vi "batch-averager-deep.vi"() -> ()   [LabVIEW 2026]
doc: "Classic LabVIEW state machine in the NI canonical form (as exported from examples/Design Patterns/State Machine/State Machine Fundamentals.vi): an inline enum type uint16{Init,Load,Accumulate,Report,Stop} carries the state through a shift register; a Case Structure inside a While loop selects the frame by that state; each frame computes the next state (a constant, or a Select between two state constants when the transition is conditional) and writes every data register through a per-frame case Out tunnel, which is the per-state multiplexer for the register value. The Stop frame is the only one that raises the stop flag through a conditional (cond=true) tunnel wired straight to the loop condition. States: Init resets the registers; Load takes the next item from Items; Accumulate adds it to the sum, advances the index and branches back to Load or on to Report by comparing the index against the item count; Report divides sum by count into the average; Stop ends the loop. Every visited state is appended to a transition Log string register. Initial State accepts any state item so the machine can start mid-sequence."
panel:
  out "Log":string
  out "Average":dbl
  out "Items Processed":i32
  out "Sum":dbl
  out "Final State":T1(ring)
  in  "Items":dbl[](array[numeric])=[1.5, 2.5, 3.5, 4.5]
  in  "Initial State":T1(ring)
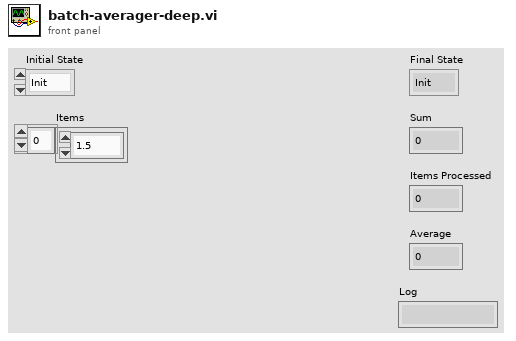
[diagram p1: front panel]
types:
  T1 = enum16{"Init", "Load", "Accumulate", "Report", "Stop"}
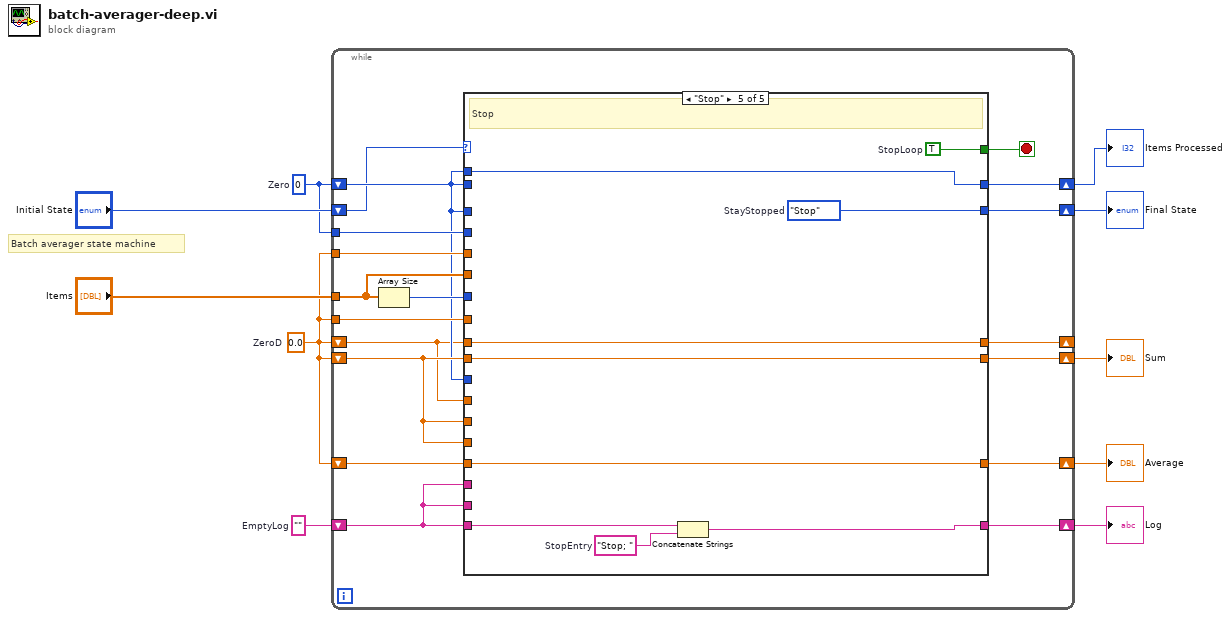
[diagram p0: block diagram]
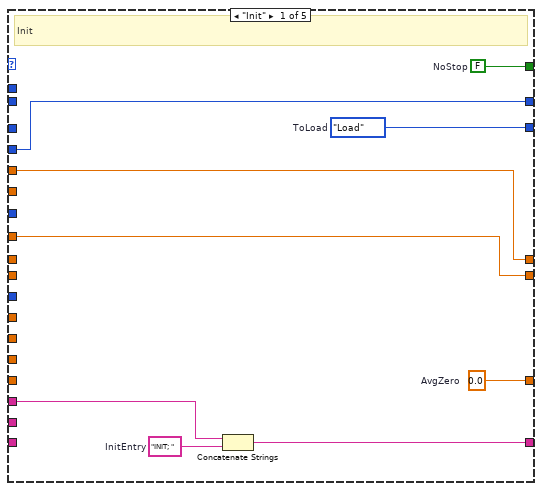
[diagram p2: hidden frame]
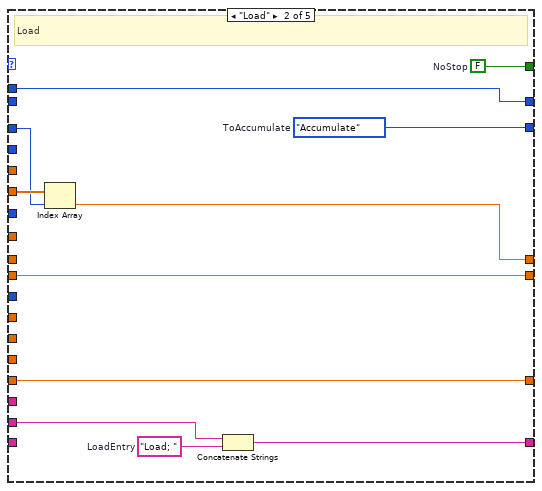
[diagram p3: hidden frame]
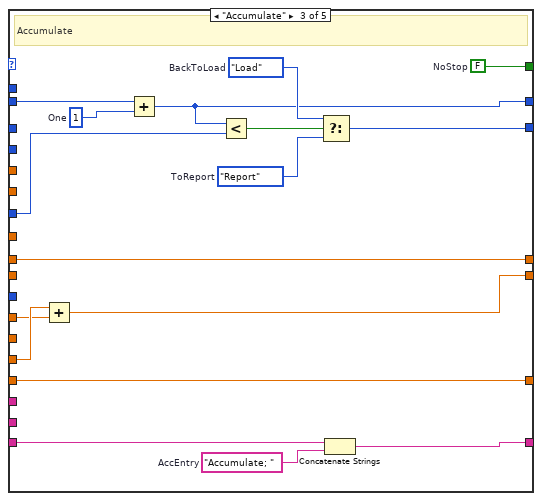
[diagram p4: hidden frame]
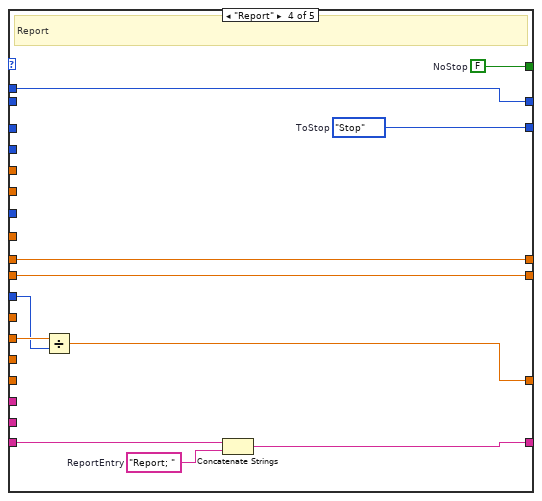
[diagram p5: hidden frame]
diagram:
  w8 = ""  # EmptyLog
  w6 = 0.0  # ZeroD
  w7 = 0  # Zero
  # "Batch averager state machine"
  n1 = while {
    tunnel: "Items" -> [w18]
    shift-right: [w28] -> w5
    shift-left: "Initial State" -> [w11]
    shift-right: [w26] -> w4
    shift-left: w6 -> [w15]
    shift-right: [w25] -> w3
    shift-left: w7 -> [w14]
    shift-right: [w24] -> _
    shift-left: w6 -> [w13]
    shift-right: [w23] -> w1
    shift-left: w8 -> [w16]
    shift-right: [w22] -> w2
    shift-left: w6 -> [w12]
    tunnel: w6 -> [w21]
    tunnel: w7 -> [w20]
    tunnel: w6 -> [w19]
    stop <- w27 stop-if-true
    n2 = Array Size(array=w18) -> (size(s)=w17:i32)
    n3 = case shown="\"Stop\"" w11 {
      tunnel: [w37 w46 w57 w74 w85] -> w28
      tunnel: [w36 w45 w56 w73 w84] -> w27
      tunnel: [w32 w41 w52 w69 w80] -> w26
      tunnel: [w31 w40 w51 w68 w79] -> w25
      tunnel: [w30 w39 w50 w67 w78] -> w24
      tunnel: [w33 w42 w53 w70 w81] -> w23
      tunnel: [w29 w38 w49 w66 w77] -> w22
      tunnel: w16 -> [w35 _ _ _ _]
      tunnel: w21 -> [w32 _ _ _ _]
      tunnel: w20 -> [w31 _ _ _ _]
      tunnel: w19 -> [w30 _ _ _ _]
      tunnel: w18 -> [_ w48 _ _ _]
      tunnel: w14 -> [_ w47 _ _ _]
      tunnel: w16 -> [_ w44 _ _ _]
      tunnel: w15 -> [_ _ w65 _ _]
      tunnel: w13 -> [_ _ w64 _ _]
      tunnel: w14 -> [_ _ w63 _ _]
      tunnel: w17 -> [_ _ w61 _ _]
      tunnel: w15 -> [_ _ _ w76 _]
      tunnel: w14 -> [_ _ _ w75 _]
      tunnel: w16 -> [_ _ w55 w72 w83]
      tunnel: w15 -> [_ w41 _ w69 w80]
      tunnel: w14 -> [_ w40 _ w68 w79]
      tunnel: w13 -> [_ _ w50 w67 w78]
      tunnel: w12 -> [_ w38 w49 _ w77]
      frame "Init" {
        w29 = 0.0  # AvgZero
        w34 = "INIT; "  # InitEntry
        w36 = FALSE  # NoStop
        w37 = T1."Load"  # ToLoad
        # "Init"
        n4 = Concatenate Strings(w35, w34) -> (w33:string)
      }
      frame "Load" {
        w43 = "Load; "  # LoadEntry
        w45 = FALSE  # NoStop
        w46 = T1."Accumulate"  # ToAccumulate
        # "Load"
        n5 = Index Array(array=w48, index=w47) -> (element=w39:dbl)
        n6 = Concatenate Strings(w44, w43) -> (w42:string)
      }
      frame "Accumulate" {
        w54 = "Accumulate; "  # AccEntry
        w56 = FALSE  # NoStop
        w58 = T1."Report"  # ToReport
        w60 = T1."Load"  # BackToLoad
        w62 = 1  # One
        # "Accumulate"
        n7 = Add(x=w65, y=w64) -> (x+y=w52:dbl)
        n8 = Add(x=w63, y=w62) -> (x+y=w51:i32)
        n9 = Less?(x=w51, y=w61) -> (x < y?=w59:bool)
        n10 = Select(t=w60, s=w59, f=w58) -> (s? t:f=w57:T1)
        n11 = Concatenate Strings(w55, w54) -> (w53:string)
      }
      frame "Report" {
        w71 = "Report; "  # ReportEntry
        w73 = FALSE  # NoStop
        w74 = T1."Stop"  # ToStop
        # "Report"
        n12 = Divide(x=w76, y=w75) -> (x/y=w66:dbl)
        n13 = Concatenate Strings(w72, w71) -> (w70:string)
      }
      frame "Stop" {
        w82 = "Stop; "  # StopEntry
        w84 = TRUE  # StopLoop
        w85 = T1."Stop"  # StayStopped
        # "Stop"
        n14 = Concatenate Strings(w83, w82) -> (w81:string)
      }
    }
  }
  "Final State" <- w5
  "Sum" <- w4
  "Items Processed" <- w3
  "Average" <- w2
  "Log" <- w1
